vi "Open Search Results Dialog.vi"(8 "error in (no error)":errorcluster, 9 "Callers":T2, 10 "State":string, 11 "Calling VI Details":T1) -> (0 "error out":errorcluster)   [LabVIEW 2020]
uses:
  JKI State Machine API/source/Support/State Calls Array.ctl
  JKI State Machine API/source/Support/State Call Cluster.ctl
  synchronization/synchronization.lvclass
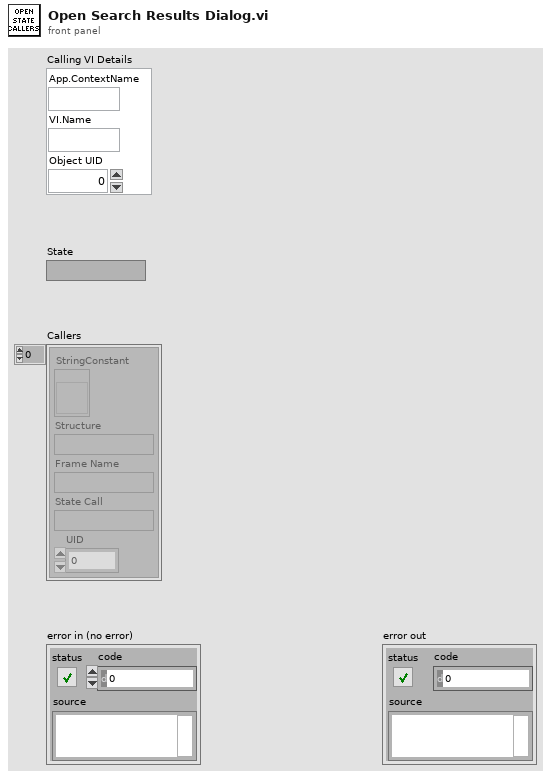
[diagram p1: front panel]
types:
  T1 = cluster{"App.ContextName":string, "VI.Name":string, "Object UID":i32}
  T2 = typedef "State Calls Array.ctl" = T3[]
  T3 = typedef "State Call Cluster.ctl" = cluster{"StringConstant":refnum<vi>, "Structure":string, "Frame Name":string, "State Call":string, "UID":i32}
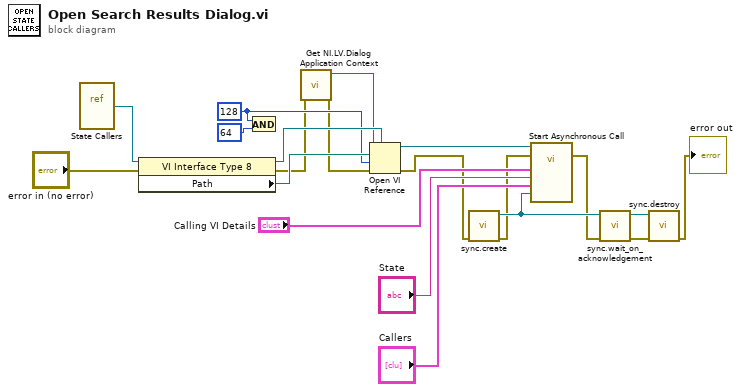
[diagram p0: block diagram]
diagram:
  w12 = 128 ("options")
  n1 = vi-ref "State Callers.vi"() -> (w20:refnum<vi>)
  n2 = property class="VI Interface Type 8"(reference=w20, error in="error in (no error)") -> (reference out=w16:refnum<vi>, error out=w11:errorcluster, "Path"=w19:path)
  n3 = And(x=w12, y=64 ("options")) -> ()  [unwired: 1 out]
  n4 = call "Get NI.LV.Dialog Application Context.vi"("error in (no error)"=w11) -> ("error out"=w10:errorcluster, "Application out"=w9:refnum<vi>)  [unwired: 9 in]
  n5 = Open VI Reference(type specifier VI Refnum (for type only)=w16, application reference (local)=w9, vi path=w19, options=w12, error in (no error)=w10) -> (vi reference=w17:refnum<vi>, error out=w4:errorcluster)  [unwired: 1 out]
  n6 = call "sync.create.vi"("error in (no error)"=w4) -> ("error out"=w1:errorcluster, "synchronization"=w5:refnum<class "synchronization.lvclass">)  [unwired: 9 in]
  n7 = call-by-ref "Start Asynchronous Call"(reference=w17, error in=w1, "synchronization"=w5, "Callers"="Callers", "State"="State", "Calling VI Details"="Calling VI Details") -> (error out=w3:errorcluster)  [unwired: 7 in, 2 out]
  n8 = call "sync.wait_on_acknowledgement.vi"("error in (no error)"=w3, "synchronization in"=w5) -> ("error out"=w6:errorcluster, "synchronization out"=w7:refnum<class "synchronization.lvclass">)  [unwired: 8 in]
  n9 = call "sync.destroy.vi"("error in (no error)"=w6, "synchronization"=w7) -> ("error out"=→"error out":errorcluster)  [unwired: 9 in]
